vi "Watchdog Reset.vi"(4 "error in (no error)":errorcluster, 7 "watchdogID in":u64 format="%.0x") -> (0 "error out":errorcluster, 3 "watchdogID out":u64 format="%.0x")   [LabVIEW 2025]
doc: "<p>Resets the <a href=\"nihelplauncher://docs/csh?context=lvrt_lvrtconcepts_rt_watchdog\">watchdog hardware</a> and associated attributes and actions to the default power-on state.</p>"
uses:
  niwd4c.dll
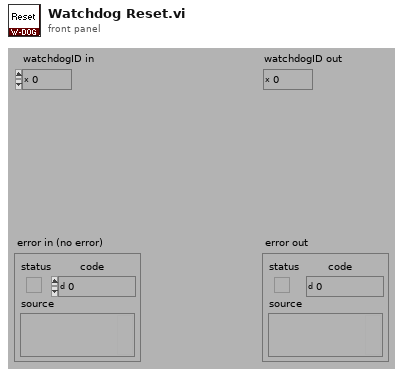
[diagram p1: front panel]
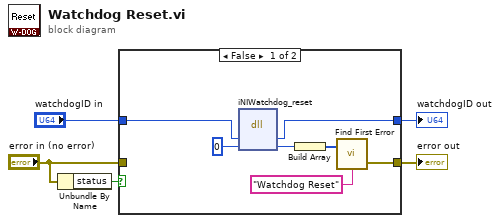
[diagram p0: block diagram]
diagram:
  n1 = Unbundle By Name("error in (no error)") -> ("status"=w5:bool)
  n2 = case shown="False" w5 {
    tunnel: [w11 w13] -> w3
    tunnel: [w6 w14] -> w4
    tunnel: "error in (no error)" -> [_ w14]
    tunnel: "watchdogID in" -> [w12 w13]
    frame False {
      n3 = dll-call lib="niwd4c.*" fn="iNIWatchdog_reset" label="Reset"("wd"=w12, "status"=0) -> ("wd"=w11:u64, "status"=w7:i32)  [unwired: 4 in, 2 out]
      n4 = Build Array(w7) -> (w9:i32[])
      n5 = call <vilib>:"Find First Error.vi"("source messages"="Watchdog Reset", "error codes"=w9) -> ("error out"=w6:errorcluster)  [unwired: 2 in, 1 out]
    }
    frame True {
    }
  }
  "error out" <- w4
  "watchdogID out" <- w3
